vi "Recall Param.vi"(8 "error in (no error)":errorcluster caption="에러 입력(에러 없음)", 10 "Recall Name":string, 11 "Instrument Manager 입력":refnum<class "Instrument Manager.lvclass">) -> (0 "error out":errorcluster caption="에러 출력", 2 "Connected?":bool, 3 "Instrument Manager 출력":refnum<class "Instrument Manager.lvclass">)   [LabVIEW 2023, in "Instrument Manager.lvclass"]
uses:
  Instrument Manager.lvclass
  Instrument Manager.lvclass/Instrument Manager.ctl
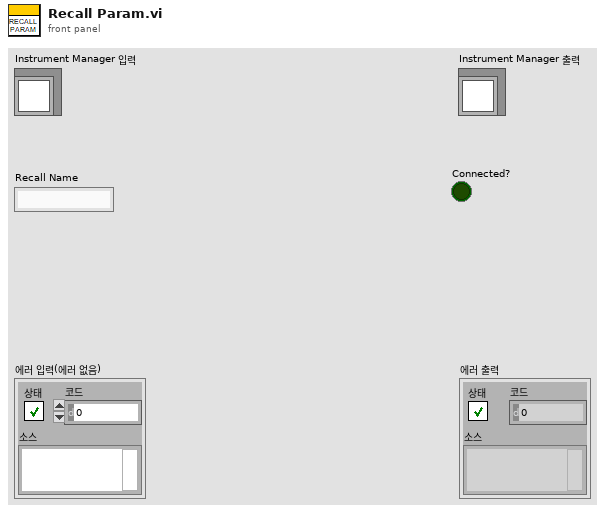
[diagram p1: front panel]
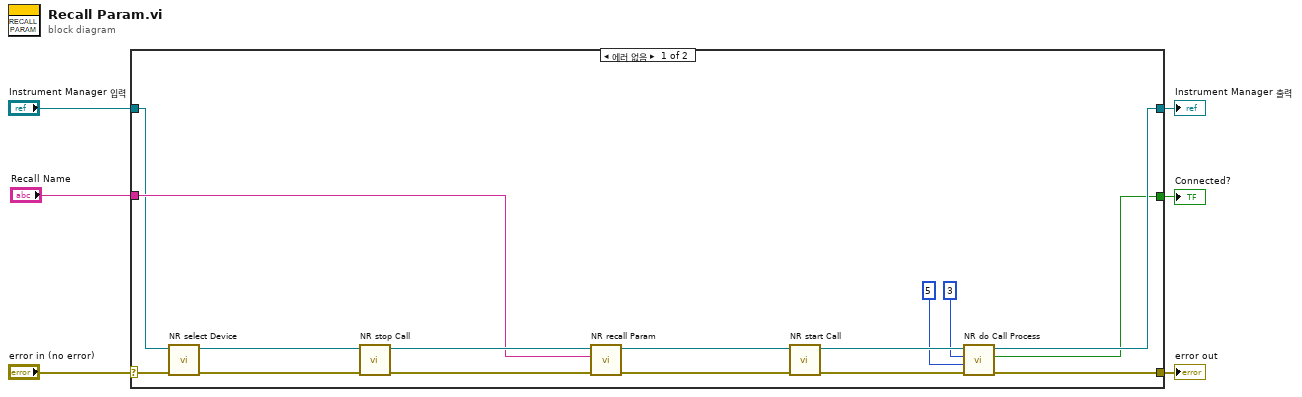
[diagram p0: block diagram]
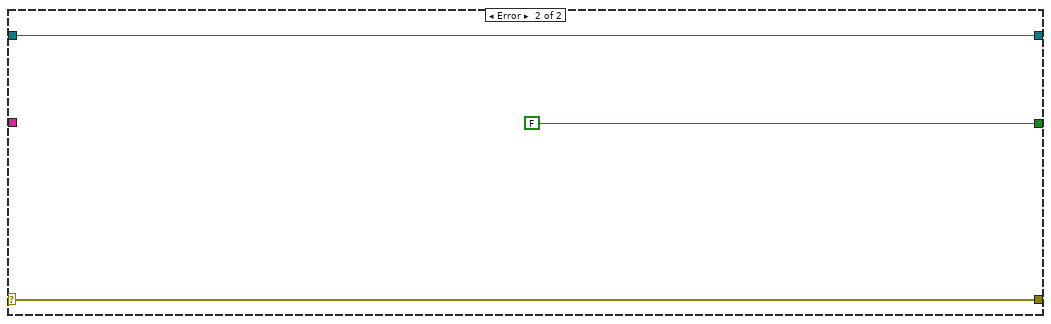
[diagram p2: hidden frame]
diagram:
  n1 = case shown="에러 없음" "error in (no error)" {
    selector: "error in (no error)" -> [w10 w25]
    tunnel: [w16 w25] -> w5
    tunnel: [w15 w24] -> w3
    tunnel: "Instrument Manager 입력" -> [w8 w24]
    tunnel: "Recall Name" -> [w18 _]
    tunnel: [w13 FALSE ("Connected?")] -> w1
    frame No Error {
      n2 = call "NR select Device.vi"("error in (no error)"=w10, "Instrument Manager 입력"=w8) -> ("error out"=w9:errorcluster, "Instrument Manager 출력"=w7:refnum<class "Instrument Manager.lvclass">)  [unwired: 8 in]
      n3 = call "NR stop Call.vi"("error in (no error)"=w9, "Instrument Manager 입력"=w7) -> ("error out"=w22:errorcluster, "Instrument Manager 출력"=w20:refnum<class "Instrument Manager.lvclass">)  [unwired: 8 in]
      n4 = call "NR recall Param.vi"("error in (no error)"=w22, "Recall Name"=w18, "Instrument Manager 입력"=w20) -> ("error out"=w21:errorcluster, "Instrument Manager 출력"=w19:refnum<class "Instrument Manager.lvclass">)  [unwired: 7 in]
      n5 = call "NR start Call.vi"("error in (no error)"=w21, "Instrument Manager 입력"=w19) -> ("error out"=w17:errorcluster, "Instrument Manager 출력"=w14:refnum<class "Instrument Manager.lvclass">)  [unwired: 8 in]
      n6 = call "NR do Call Process.vi"("error in (no error)"=w17, "Waiting Time"=5, "Max Retry Count"=3, "Instrument Manager 입력"=w14) -> ("error out"=w16:errorcluster, "Connected?"=w13:bool, "Instrument Manager 출력"=w15:refnum<class "Instrument Manager.lvclass">)  [unwired: 5 in]
    }
    frame Error {
    }
  }
  "error out" <- w5
  "Instrument Manager 출력" <- w3
  "Connected?" <- w1
